vi "Launch DAQ Interface.vi"(8 "error in (no error)":errorcluster, 11 "Guardian in":refnum<class "Guardian.lvclass">) -> (0 "error out":errorcluster, 3 "Guardian out":refnum<class "Guardian.lvclass">)   [LabVIEW 2020, in "TALOS.lvlib" / "Guardian.lvlib" / "Guardian.lvclass"]
uses:
  Guardian.lvclass
  C:/Users/marco/Documents/GitHub_Lab/TALOS/talos/Ancestor/Ancestor/Ancestor.lvclass
  C:/Users/marco/Documents/GitHub_Lab/TALOS/builds/Actor Framework PPL/Actor Framework.lvlibp/1abvi3w/vi.lib/ActorFramework/Actor/Actor.lvclass
  Ancestor/Ancestor/Ancestor.lvclass/Ancestor.ctl
  Guardian Messages/Launch uService Msg/Launch uService Msg.lvclass/Launch uService Msg.ctl
  Ancestor/Ancestor/Read ID.vi
  Support VIs/Global Memory.vi
  builds/Actor Framework PPL/Actor Framework.lvlibp/1abvi3w/vi.lib/ActorFramework/Message Enqueuer/Enqueue.vi
  Guardian Messages/Launch uService Msg/Launch uService Msg.lvclass
  Guardian.lvclass/Guardian.ctl
  builds/Actor Framework PPL/Actor Framework.lvlibp/1abvi3w/vi.lib/ActorFramework/Actor/Actor.lvclass
  TALOS.lvlib
  C:/Users/marco/Documents/GitHub_Lab/TALOS/talos/Guardian/Guardian/Guardian.lvclass
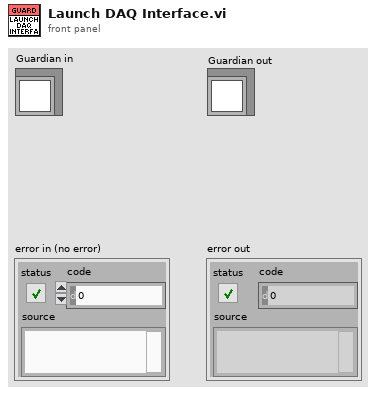
[diagram p1: front panel]
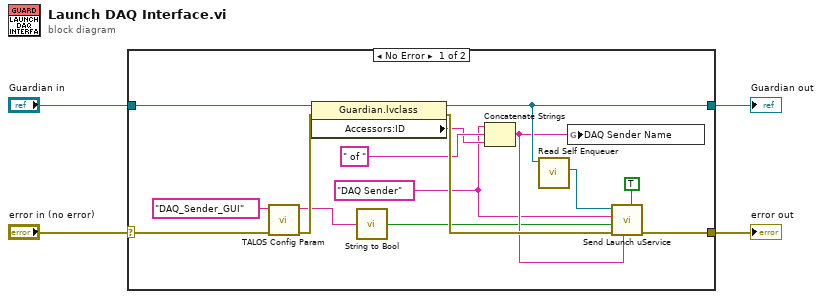
[diagram p0: block diagram]
diagram:
  n1 = case shown="No Error" "error in (no error)" {
    selector: "error in (no error)" -> [w9 w21]
    tunnel: "Guardian in" -> [w16 w20]
    tunnel: [w18 w21] -> w2
    tunnel: [w14 w20] -> w1
    frame No Error {
      w10 = "DAQ Sender"
      n2 = call "TALOS Config Param.vi"("error in (no error)"=w9, "Parameter Name"="DAQ_Sender_GUI") -> ("error out"=w8:errorcluster, "Output"=w6:string)  [unwired: 8 in]
      n3 = property class="Guardian.lvclass"(reference=w16, error in=w8) -> (reference out=w14:refnum<class "Guardian.lvclass">, error out=w15:errorcluster, "Accessors:ID"=w12:string)
      n4 = call "String to Bool.vi"("String"=w6) -> ("Boolean"=w5:bool)
      n5 = Concatenate Strings(w10, " of ", w12) -> (w11:string)
      n6 = call "Read Self Enqueuer.vi"("Actor"=w14) -> ("Self Enqueuer"=w19:refnum<class "Message Enqueuer.lvclass">)  [unwired: 10 in]
      n7 = global write "Global Memory.vi" "DAQ Sender Name"(w11) -> ()
      n8 = call "Send Launch uService.vi"("Highlander?"=TRUE, "uService ID"=w11, "error in (no error)"=w15, "GUI?"=w5, "uService Class Name"=w10, "Message Enqueuer"=w19) -> ("error out"=w18:errorcluster)  [unwired: 4 in, 1 out]
    }
    frame Error {
    }
  }
  "error out" <- w2
  "Guardian out" <- w1
